vi "Initialize Joystick.vi"(8 "error in (no error)":errorcluster, 11 "device index":i32) -> (0 "error out":errorcluster, 2 "return type":i32, 3 "device ID":refnum<k1>)   [LabVIEW 2026]
doc: "<p>Opens a reference to and initializes a joystick device at the index you specify.</p>"
uses:
  LabVIEW Data/libDS4LabVIEW.dylib
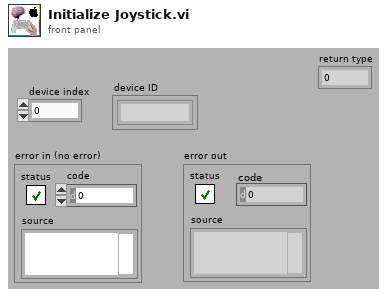
[diagram p1: front panel]
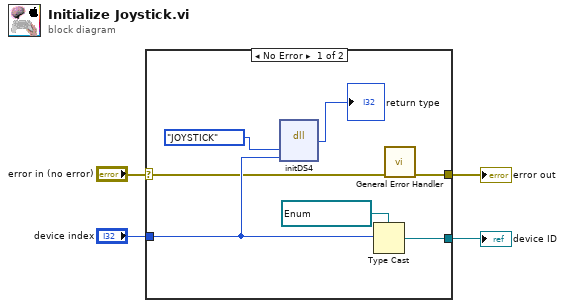
[diagram p0: block diagram]
diagram:
  n1 = case shown="No Error" "error in (no error)" {
    selector: "error in (no error)" -> [w6 w12]
    tunnel: [w7 w12] -> w4
    tunnel: "device index" -> [w9 _]
    tunnel: [w8 _] -> w1
    frame No Error {
      w11 = refnum<k1> refnum items=["JOYSTICK"] ("JOYSTICK")
      n2 = dll-call lib="Users/eira/Documents/LabVIEW Data/libDS4LabVIEW.dylib" fn="initDS4"(enum16{"JOYSTICK", "KEYBOARD", "MOUSE"}."JOYSTICK" ("Enum"), w9) -> ("return type"=→"return type":i32)  [unwired: 5 in, 2 out]
      n3 = Type Cast(type=w11, x=w9) -> (*(type *) &x=w8:refnum<k1>)
      n4 = call <vilib>:"General Error Handler.vi"("error in (no error)"=w6) -> ("error out"=w7:errorcluster)  [unwired: 10 in, 4 out]
    }
    frame Error {
    }
  }
  "error out" <- w4
  "device ID" <- w1
